vi "Create Test Configuration.vi"() -> (0 "error out":errorcluster, 1 "Names":string[](array[string]), 2 "Line Array":T1[](array[typedef]), 3 "Module Configuration":refnum<class "PID Module configuration.lvclass">, 4 "Channels":refnum<class "TBM channel.lvclass">[](array[class]), 5 "instance identifier":string)   [LabVIEW 2015, in "PID Module tests.lvlib"]
doc: "This VI creates a standard test configuration for other unit tests. It currently creates and adds one line with every datatype to the module configuration."
uses:
  PID Module tests.lvlib
  module/configuration/PID Module configuration.lvclass
  module/configuration/Line.ctl
  <vilib>/NI/Tag Bus Module Framework/channel/TBM channel.lvclass
  <vilib>/NI/Tag Bus/tag/tag descriptor.lvclass/tag descriptor.ctl
  <vilib>/NI/Tag Bus/tag/default value polymorphs/write default value Double.vi
  <vilib>/NI/Configuration Framework/serializable configuration/NISE_CEF_serializable configuration.lvclass
  <vilib>/NI/Tag Bus/tag/tag descriptor.lvclass
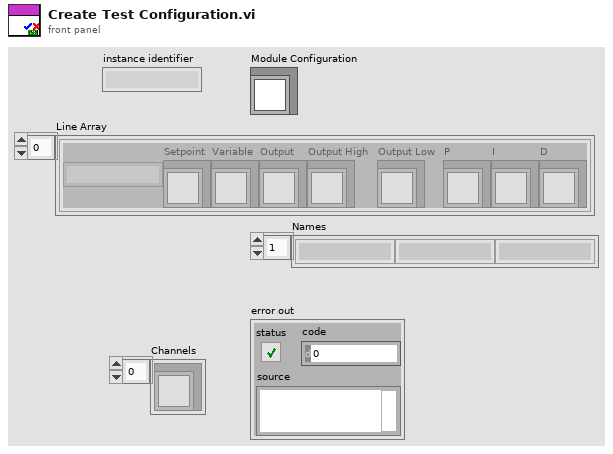
[diagram p1: front panel]
types:
  T1 = typedef "PID Module configuration.lvclass/Line.ctl" = cluster{"PID ID":string, "Setpoint":refnum<class "TBM channel.lvclass">, "Variable":refnum<class "TBM channel.lvclass">, "Output":refnum<class "TBM channel.lvclass">, "Output High":refnum<class "TBM channel.lvclass">, "Output Low":refnum<class "TBM channel.lvclass">, "P":refnum<class "TBM channel.lvclass">, "I":refnum<class "TBM channel.lvclass">, "D":refnum<class "TBM channel.lvclass">}
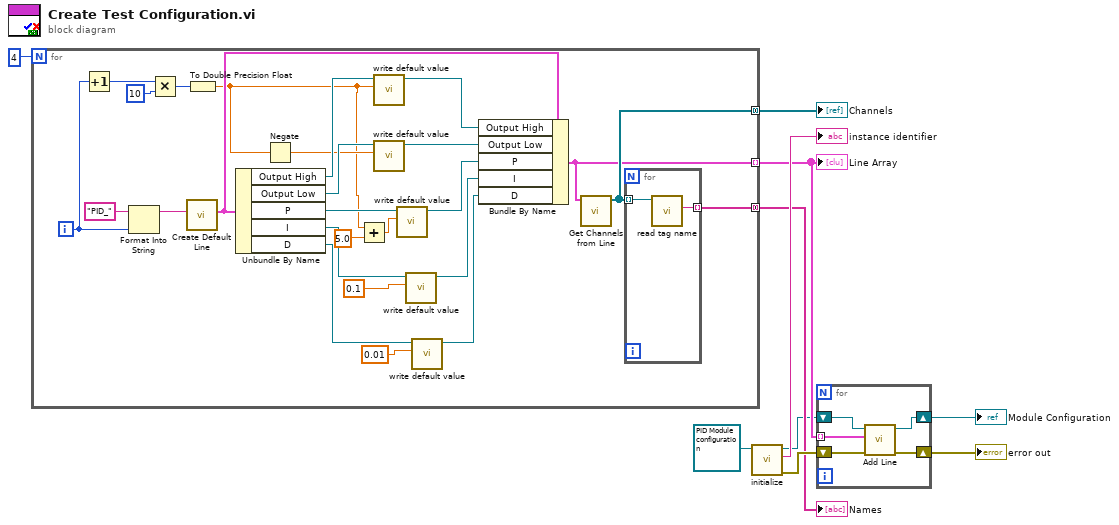
[diagram p0: block diagram]
diagram:
  n1 = for {
    N: 4 -> [_]
    tunnel: [w24] -> w6 mode=indexing
    tunnel: [w35] -> w2 mode=concatenating
    tunnel: [w34] -> w7 mode=concatenating
    i -> [w31]
    n2 = Increment(x=w31) -> (x+1=w30:i32)
    n3 = Format Into String(initial string="PID_", w31) -> (resulting string=w33:string)  [unwired: 2 in, 1 out]
    n4 = Multiply(x=w30, y=10) -> (x*y=w22:i32)
    n5 = call "Create Default Line.vi"("Line Name"=w33) -> ("Default Line"=w32:T1)  [unwired: 10 in]
    n6 = To Double Precision Float(number=w22) -> (double precision float=w12:dbl)
    n7 = Unbundle By Name(w32) -> ("Output High"=w25:refnum<class "TBM channel.lvclass">, "Output Low"=w28:refnum<class "TBM channel.lvclass">, "P"=w21:refnum<class "TBM channel.lvclass">, "I"=w19:refnum<class "TBM channel.lvclass">, "D"=w15:refnum<class "TBM channel.lvclass">)
    n8 = Negate(x=w12) -> (-x=w23:dbl)
    n9 = Add(x=w12, y=5.0 ("default value")) -> (x+y=w13:dbl)
    n10 = call-poly <vilib>:"write default value.vi"("default value"=w12, "system tag in"=w25) -> ("system tag out"=w26:refnum<class "TBM channel.lvclass">)  [unwired: 8 in, 1 out]
    n11 = call-poly <vilib>:"write default value.vi"("default value"=w23, "system tag in"=w28) -> ("system tag out"=w27:refnum<class "TBM channel.lvclass">)  [unwired: 8 in, 1 out]
    n12 = call-poly <vilib>:"write default value.vi"("default value"=w13, "system tag in"=w21) -> ("system tag out"=w20:refnum<class "TBM channel.lvclass">)  [unwired: 8 in, 1 out]
    n13 = call-poly <vilib>:"write default value.vi"("default value"=0.1, "system tag in"=w19) -> ("system tag out"=w18:refnum<class "TBM channel.lvclass">)  [unwired: 8 in, 1 out]
    n14 = call-poly <vilib>:"write default value.vi"("default value"=0.01, "system tag in"=w15) -> ("system tag out"=w14:refnum<class "TBM channel.lvclass">)  [unwired: 8 in, 1 out]
    n15 = Bundle By Name(cluster=w32, "Output High"=w26, "Output Low"=w27, "P"=w20, "I"=w18, "D"=w14) -> (w24:T1)
    n16 = call "Get Channels from Line.vi"("Line"=w24) -> ("Channels"=w35:refnum<class "TBM channel.lvclass">[])  [unwired: 10 in]
    n17 = for {
      tunnel: w35 -> [w38] mode=indexing
      tunnel: [w37] -> w34 mode=indexing
      n18 = call <vilib>:"read tag name.vi"("system tag in"=w38) -> ("name"=w37:string)  [unwired: 8 in, 2 out]
    }
  }
  "Names" <- w7
  "Line Array" <- w6
  "Channels" <- w2
  n19 = call <vilib>:"initialize.vi"("configuration in"=refnum<class "PID Module configuration.lvclass"> refnum ("tag bus configurable plugin module configuration")) -> ("error out"=w8:errorcluster, "identifier"=→"instance identifier":string, "configuration out"=w3:refnum<class "PID Module configuration.lvclass">)  [unwired: 8 in]
  n20 = for {
    tunnel: w6 -> [w39] mode=indexing
    shift-right: [w42] -> w5
    shift-left: w3 -> [w43]
    shift-right: [w40] -> w10
    shift-left: w8 -> [w41]
    n21 = call "Add Line.vi"("error in"=w41, "Line"=w39, "PID Module configuration in"=w43) -> ("error out"=w40:errorcluster, "PID Module configuration out"=w42:refnum<class "PID Module configuration.lvclass">)  [unwired: 6 in, 1 out]
  }
  "error out" <- w10
  "Module Configuration" <- w5
